vi "Find Tagged and Wire.vi"(6 "TagName":string="phygbuTag", 7 "RegExp Search?":bool, 8 "error in (no error)":errorcluster, 9 "TagValue":string, 10 "Single Reference":refnum<vi>, 11 "Multiple  References":refnum<vi>[](array[refnum])) -> (0 "error out":errorcluster, 3 "Found Terminal":refnum<vi>)   [LabVIEW 2012, in "Scripting Tools.lvlib"]
doc: "Find a reference in the Multiple References array that is tagged with the given tag and value and wire the first terminal associated with that object to the first terminal associated with the Single reference. returns a reference to the first terminal of the tagged object if found, or not a reference if not found."
uses:
  Scripting Tools.lvlib
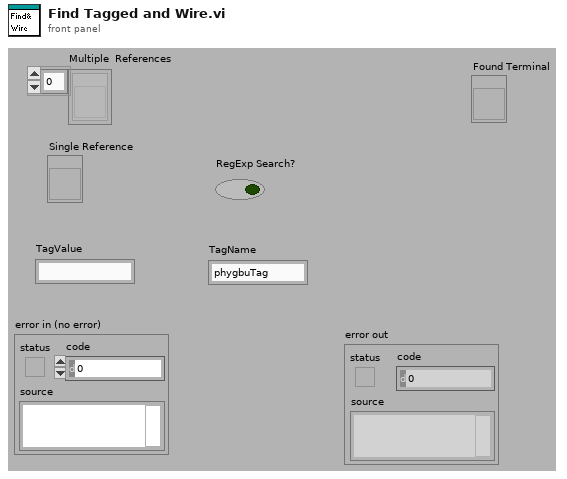
[diagram p1: front panel]
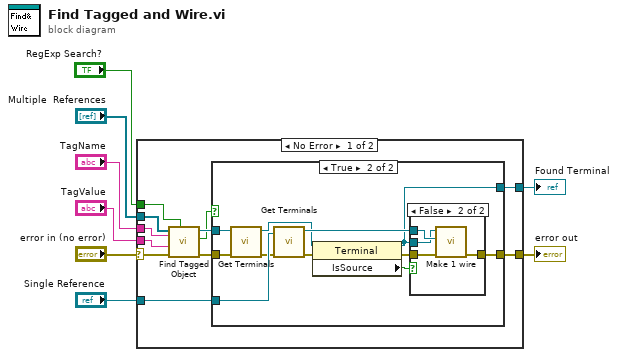
[diagram p0: block diagram]
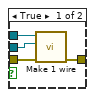
[diagram p3: hidden frame]
diagram:
  n1 = case shown="No Error" "error in (no error)" {
    selector: "error in (no error)" -> [w9 w40]
    tunnel: "Multiple  References" -> [w19 _]
    tunnel: "RegExp Search?" -> [w18 _]
    tunnel: "TagValue" -> [w17 _]
    tunnel: "TagName" -> [w16 _]
    tunnel: "Single Reference" -> [w14 _]
    tunnel: [w11 w40] -> w3
    tunnel: [w10 _] -> w2
    frame No Error {
      n2 = call "Find Tagged Object.vi"("RegExp Search?"=w18, "error in (no error)"=w9, "TagValue"=w17, "TagName"=w16, "Array of References"=w19) -> ("error out"=w12:errorcluster, "Found?"=w13:bool, "reference"=w15:refnum<vi>)  [unwired: 4 out]
      n3 = case shown="True" w13 {
        tunnel: w15 -> [_ w31]
        tunnel: w14 -> [_ w30]
        tunnel: w12 -> [w20 w25]
        tunnel: [w20 w28] -> w11
        tunnel: [_ w21] -> w10
        frame False {
        }
        frame True {
          n4 = call "Get Terminals.vi"("error in (no error)"=w25, "Reference"=w31) -> ("error out"=w24:errorcluster, "First Terminal"=w27:refnum<vi>)  [unwired: 8 out]
          n5 = call "Get Terminals.vi"("error in (no error)"=w24, "Reference"=w30) -> ("error out"=w23:errorcluster, "First Terminal"=w29:refnum<vi>)  [unwired: 8 out]
          n6 = property on="Property Node" class="Terminal"(reference=w27, error in=w23) -> (reference out=w21:refnum<vi>, error out=w22:errorcluster, "IsSource"=w26:bool)
          n7 = case shown="False" w26 {
            tunnel: w29 -> [w32 w37]
            tunnel: w22 -> [w35 w39]
            tunnel: [w34 w38] -> w28
            tunnel: w21 -> [w33 w36]
            frame True {
              n8 = call "Make 1 wire.vi"("error in"=w35, "Wire Terminal 2"=w33, "Wire Terminal 1"=w32) -> ("error out"=w34:errorcluster)  [unwired: 8 out]
            }
            frame False {
              n9 = call "Make 1 wire.vi"("error in"=w39, "Wire Terminal 2"=w37, "Wire Terminal 1"=w36) -> ("error out"=w38:errorcluster)  [unwired: 8 out]
            }
          }
        }
      }
    }
    frame Error {
    }
  }
  "error out" <- w3
  "Found Terminal" <- w2
